vi "CAN Frame Input Single Point_xjm.vi"() -> ()   [LabVIEW 2020]
doc: "This example demonstrates receiving frames using an NI-XNET Frame Input session. \n\nThis example can run against the CAN Frame Output Single Point example, assuming you have a properly terminated CAN cable connected to two CAN ports.\n\nIf you have no database aliases on your system, the example automatically loads the nixnet_example database."
uses:
  <vilib>/xnet/xnet.llb/XNET Frame CAN.ctl
  <vilib>/xnet/xnet.llb/XNET Frame Type CAN.ctl
  <vilib>/xnet/xnet.llb/XNET Create Session (Frame Input Single-point).vi
  <vilib>/xnet/xnet.llb/XNET Read (Frame CAN).vi
panel:
  out "CAN Frame Input":T1[](array[typedef]) {"payload" format="%x"; "timestamp" format="%<%.7X\n%x>T"; "type" items=["CAN Data"=0, "CAN Remote"=1, "CAN Bus Error"=2, "CAN 2.0 Data"=8, "CAN FD Data"=16, "CAN FD+BRS Data"=24, "J1939 Data"=192, "Delay"=224, "Log Trigger"=225, "Start Trigger"=226]; "identifier" format="%x"}
  in  "Select Frames":refnum<k21>[](array[refnum])=["CANEventFrame1\nnixnet_example.CAN_Cluster", "CANEventFrame2\nnixnet_example.CAN_Cluster"]
  in  "Select Interface":refnum<k21>="CAN2"
  in  "stop":bool
  # "Overview: Demonstrates the use of Frame Input Single Point XNET Sessions with a CAN interface.\nRequirements: LabVIEW, NI-XNET\nInstructions: \n1. Ensure that you are have connected the selected CAN port to another CAN interface outputting data. This example can be used with any CAN output example.\n2.  Run the VI."
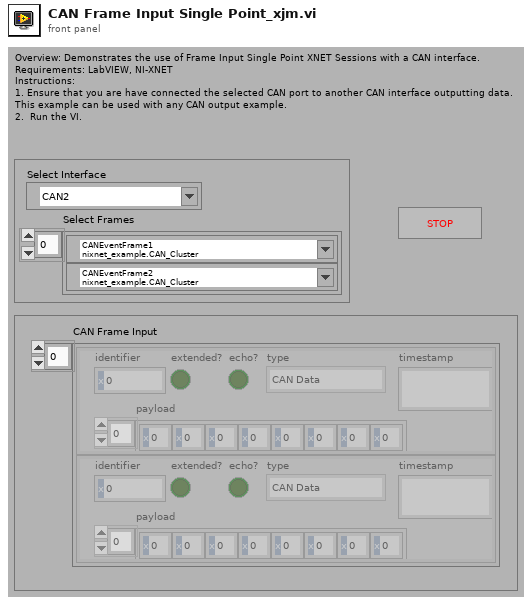
[diagram p1: front panel]
types:
  T1 = typedef "XNET Frame CAN.ctl" = cluster{"timestamp":timestamp, "payload":u8[], "identifier":u32, "type":T2, "extended?":bool, "echo?":bool}
  T2 = typedef "XNET Frame Type CAN.ctl" = u8
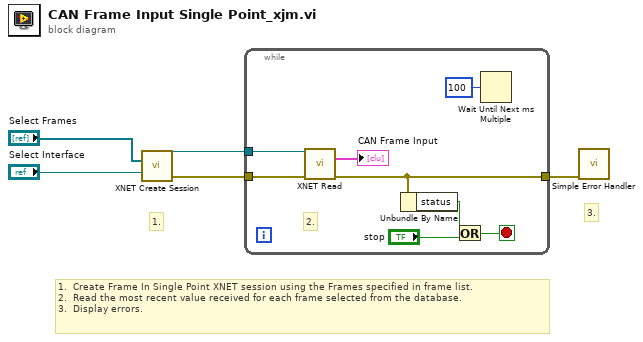
[diagram p0: block diagram]
diagram:
  # "3."
  # "1."
  # "1.  Create Frame In Single Point XNET session using the Frames specified in frame list.  \n2.  Read the most recent value received for each frame selected from the database.\n3.  Display errors."
  n1 = call-poly <vilib>:"XNET Create Session.vi"("frame list"="Select Frames", "interface"="Select Interface") -> ("session out"=w2:refnum<k21>, "error out"=w1:errorcluster)  [unwired: 1 in, 11 out]
  n2 = while {
    tunnel: w2 -> [w13]
    tunnel: w1 -> [w12]
    tunnel: [w11] -> w4
    stop <- w8 stop-if-true
    # "2."
    n3 = call-poly <vilib>:"XNET Read.vi"("session in"=w13, "error in (no error)"=w12) -> ("data"=→"CAN Frame Input":T1[], "error out"=w11:errorcluster)  [unwired: 12 out]
    n4 = Unbundle By Name(w11) -> ("status"=w10:bool)
    n5 = Or(x=w10, y="stop") -> (x .or. y?=w8:bool)
    n6 = Wait Until Next ms Multiple(millisecond multiple=u32 100 ("milliseconds to wait")) -> ()  [unwired: 1 out]
  }
  n7 = call <vilib>:"Simple Error Handler.vi"("error in (no error)"=w4) -> ()  [unwired: 1 in, 8 out]
